vi "AssertTrueOrFalse_Tests.vi"(11 "error in":errorcluster) -> (15 "error out":errorcluster)   [LabVIEW 2016, in "DronaTest.lvlib"]
uses:
  DronaTest.lvlib
  APIs/Assert/AssertControlValue/False.vi
  <vilib>/addons/_JKI Toolkits/Caraya/classes/Assert/Assert Error.vi
  <vilib>/addons/_JKI Toolkits/Caraya/classes/Assert/Assert Equal Value_Variant.vi
  APIs/Assert/AssertControlValue/True.vi
  <vilib>/addons/_JKI Toolkits/Caraya/classes/Test/Test.lvclass
  Drona.lvlib
  <vilib>/addons/_JKI Toolkits/Caraya/classes/Assert/Assert.lvclass
  APIs/Assert/AssertControlValue/AssertControlValue.lvlib
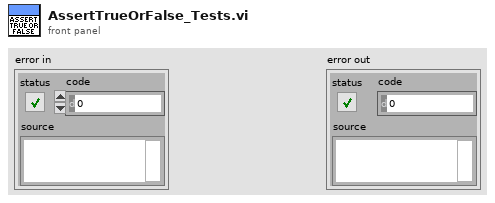
[diagram p1: front panel]
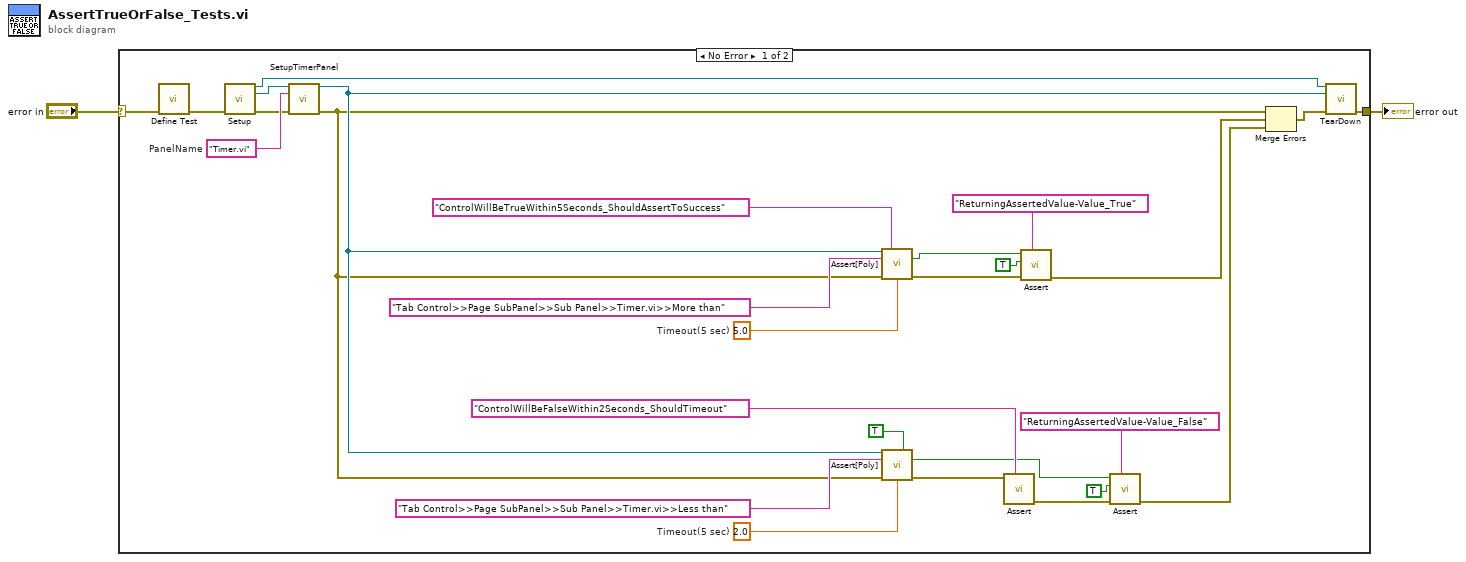
[diagram p0: block diagram]
diagram:
  n1 = case shown="No Error" "error in" {
    selector: "error in" -> [w30 w31]
    tunnel: [w16 w31] -> w1
    frame No Error {
      w22 = "Timer.vi"  # PanelName
      w26 = 2.0  # Timeout(5 sec)
      w27 = 5.0  # Timeout(5 sec)
      n2 = call <vilib>:"Define Test.vi"("error in (no error)"=w30) -> ("error out"=w19:errorcluster)  [unwired: 9 in, 1 out]
      n3 = call "Setup.vi"("error in (no error)"=w19) -> ("Application Ref"=w15:refnum<vi>, "VI out"=w20:refnum<vi>, "error out"=w21:errorcluster)  [unwired: 12 in]
      n4 = call "SetupTimerPanel.vi"("VI in"=w20, "Item Name"=w22, "error in (no error)"=w21) -> ("VI out"=w18:refnum<vi>, "error out"=w14:errorcluster)  [unwired: 11 in]
      n5 = call-poly "Assert[Poly].vi"("VI Reference In"=w18, "Test Label"="ControlWillBeTrueWithin5Seconds_ShouldAssertToSuccess" ("string"), "Control Path"="Tab Control>>Page SubPanel>>Sub Panel>>Timer.vi>>More than", "Error In"=w14, "Timeout(5 sec)"=w27) -> ("Asserted Value"=w11:bool, "Error Out"=w13:errorcluster)  [unwired: 8 in, 1 out]
      n6 = call-poly "Assert[Poly].vi"("VI Reference In"=w18, "Assert Only? (F)"=TRUE, "Control Path"="Tab Control>>Page SubPanel>>Sub Panel>>Timer.vi>>Less than", "Error In"=w14, "Timeout(5 sec)"=w26) -> ("Asserted Value"=w6:bool, "Error Out"=w9:errorcluster)  [unwired: 8 in, 1 out]
      n7 = call-poly <vilib>:"Assert.vi"("Label"="ControlWillBeFalseWithin2Seconds_ShouldTimeout" ("string"), "Error?"=w9) -> ("error out"=w4:errorcluster)  [unwired: 8 in, 1 out]
      n8 = call-poly <vilib>:"Assert.vi"("Label"="ReturningAssertedValue-Value_True", "error in (no error)"=w13, "Y"=TRUE ("Asserted Value"), "X"=w11) -> ("error out"=w12:errorcluster)  [unwired: 6 in, 1 out]
      n9 = call-poly <vilib>:"Assert.vi"("Label"="ReturningAssertedValue-Value_False", "error in (no error)"=w4, "Y"=TRUE ("Assert Only? (F)"), "X"=w6) -> ("error out"=w3:errorcluster)  [unwired: 6 in, 1 out]
      n10 = Merge Errors(w14, w12, w3) -> (w17:errorcluster)
      n11 = call "TearDown.vi"("Application Ref"=w15, "VI in"=w18, "error in (no error)"=w17) -> ("error out"=w16:errorcluster)  [unwired: 12 in]
    }
    frame Error {
    }
  }
  "error out" <- w1
